vi "Test exp fit.vi"() -> ()   [LabVIEW 2020]
uses:
  controls/Color --typedef.ctl
  <vilib>/Utility/file.llb/Read Delimited Spreadsheet (DBL).vi
panel:
  out "MSE (red)":dbl
  out "MSE (green)":dbl
  out "MSE (blue)":dbl
  out "Red":cluster{dbl[], dbl[]}[](graph)
  out "Blue":cluster{dbl[], dbl[]}[](graph)
  out "Green":cluster{dbl[], dbl[]}[](graph)
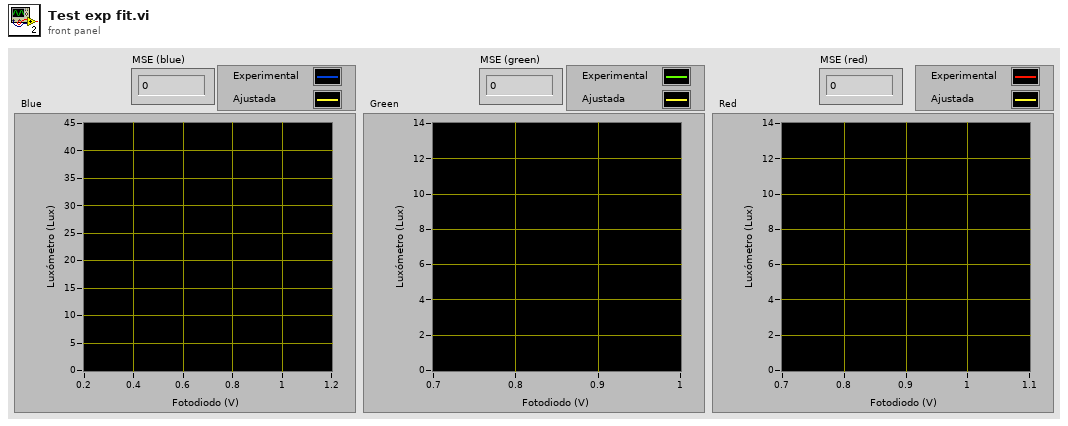
[diagram p1: front panel]
types:
  T1 = typedef "Color --typedef.ctl" = enum16{"Violeta (360-450nm)", "Azul (450-500nm)", "Verde(500-570nm)", "Amarillo (570-590nm)", "Naranja (600-610nm)", "Rojo (610-670nm)", "Blanco"}
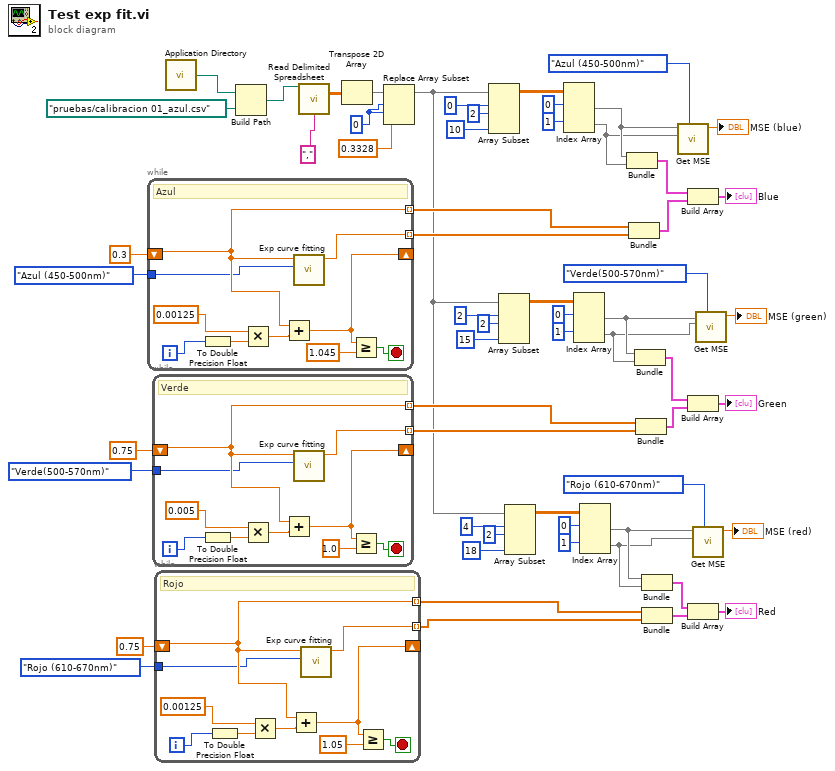
[diagram p0: block diagram]
diagram:
  w14 = 0 ("index (row)")
  n1 = while {
    shift-right: [w63] -> _
    shift-left: 0.3 -> [w62]
    tunnel: [w66] -> w55 mode=indexing
    tunnel: [w62] -> w54 mode=indexing
    tunnel: Color_--typedef."Azul (450-500nm)" ("Color 2") -> [w61]
    i -> [w70]
    stop <- w65 stop-if-true
    # "Azul"
    n2 = To Double Precision Float(number=w70) -> (double precision float=w69:dbl)
    n3 = Multiply(x=0.00125, y=w69) -> (x*y=w67:dbl)
    n4 = Add(x=w62, y=w67) -> (x+y=w63:dbl)
    n5 = call "Exp curve fitting.vi"("Color"=w61, "x (volts)"=w62) -> ("y (Lux)"=w66:dbl)  [unwired: 9 in]
    n6 = Greater Or Equal?(x=w63, y=1.045) -> (x >= y?=w65:bool)
  }
  n7 = while {
    shift-right: [w73] -> _
    shift-left: 0.75 -> [w72]
    tunnel: [w76] -> w58 mode=indexing
    tunnel: [w72] -> w59 mode=indexing
    tunnel: Color_--typedef."Verde(500-570nm)" ("Color") -> [w71]
    i -> [w80]
    stop <- w75 stop-if-true
    # "Verde"
    n8 = To Double Precision Float(number=w80) -> (double precision float=w79:dbl)
    n9 = Multiply(x=0.005, y=w79) -> (x*y=w77:dbl)
    n10 = Add(x=w72, y=w77) -> (x+y=w73:dbl)
    n11 = call "Exp curve fitting.vi"("Color"=w71, "x (volts)"=w72) -> ("y (Lux)"=w76:dbl)  [unwired: 9 in]
    n12 = Greater Or Equal?(x=w73, y=1.0) -> (x >= y?=w75:bool)
  }
  n13 = while {
    shift-right: [w83] -> _
    shift-left: 0.75 -> [w82]
    tunnel: [w86] -> w50 mode=indexing
    tunnel: [w82] -> w51 mode=indexing
    tunnel: Color_--typedef."Rojo (610-670nm)" ("Color 2") -> [w81]
    i -> [w90]
    stop <- w85 stop-if-true
    # "Rojo"
    n14 = To Double Precision Float(number=w90) -> (double precision float=w89:dbl)
    n15 = Multiply(x=0.00125, y=w89) -> (x*y=w87:dbl)
    n16 = Add(x=w82, y=w87) -> (x+y=w83:dbl)
    n17 = call "Exp curve fitting.vi"("Color"=w81, "x (volts)"=w82) -> ("y (Lux)"=w86:dbl)  [unwired: 9 in]
    n18 = Greater Or Equal?(x=w83, y=1.05) -> (x >= y?=w85:bool)
  }
  n19 = call <vilib>:"Application Directory.vi"() -> ("Application Directory"=w48:path)
  n20 = Build Path(base path=w48, name or relative path=path "pruebas/calibracion 01_azul.csv") -> (appended path=w46:path)
  n21 = call-poly <vilib>:"Read Delimited Spreadsheet.vi"("file path (dialog if empty)"=w46, "delimiter (\\t)"="," ("delimiter (\\t)")) -> ("all rows"=w16:dbl[][])  [unwired: 8 in, 5 out]
  n22 = Transpose 2D Array(2D array=w16) -> (transposed array=w20:dbl[][])
  n23 = Replace Array Subset(array=w20, new element=0.3328 ("new element/subarray"), index (row)=w14, index (col)=w14) -> (w15:dbl[][])
  n24 = Array Subset(array=w15, index (row)=0 ("index"), length (row)=2 ("length"), length (col)=10 ("length")) -> (w44:dbl[][])  [unwired: 1 in]
  n25 = Array Subset(array=w15, index (row)=2 ("index"), length (row)=2 ("length"), length (col)=15 ("length")) -> (w30:dbl[][])  [unwired: 1 in]
  n26 = Array Subset(array=w15, index (row)=4 ("index"), length (row)=2 ("length"), length (col)=18 ("length")) -> (w26:dbl[][])  [unwired: 1 in]
  n27 = Index Array(array=w44, index (row) #1=0 ("index (row)"), index (row) #2=1 ("index (row)")) -> (element #1=w12:dbl[], element #2=w8:dbl[])  [unwired: 2 in]
  n28 = Index Array(array=w30, index (row) #1=0 ("index (row)"), index (row) #2=1 ("index (row)")) -> (element #1=w9:dbl[], element #2=w7:dbl[])  [unwired: 2 in]
  n29 = Index Array(array=w26, index (row) #1=0 ("index (row)"), index (row) #2=1 ("index (row)")) -> (element #1=w3:dbl[], element #2=w2:dbl[])  [unwired: 2 in]
  n30 = Bundle(w12, w8) -> (w38:cluster{dbl[], dbl[]})  [unwired: 1 in]
  n31 = Bundle(w54, w55) -> (w37:cluster{dbl[], dbl[]})  [unwired: 1 in]
  n32 = Bundle(w9, w7) -> (w29:cluster{dbl[], dbl[]})  [unwired: 1 in]
  n33 = Bundle(w59, w58) -> (w28:cluster{dbl[], dbl[]})  [unwired: 1 in]
  n34 = Bundle(w3, w2) -> (w19:cluster{dbl[], dbl[]})  [unwired: 1 in]
  n35 = Bundle(w51, w50) -> (w18:cluster{dbl[], dbl[]})  [unwired: 1 in]
  n36 = call "Get MSE.vi"("Color"=Color_--typedef."Azul (450-500nm)", "y (lux)"=w8, "x (volts)"=w12) -> ("MSE"=→"MSE (blue)":dbl)  [unwired: 8 in]
  n37 = Build Array(w38, w37) -> (→"Blue":cluster{dbl[], dbl[]}[])
  n38 = Build Array(w29, w28) -> (→"Green":cluster{dbl[], dbl[]}[])
  n39 = Build Array(w19, w18) -> (→"Red":cluster{dbl[], dbl[]}[])
  n40 = call "Get MSE.vi"("Color"=Color_--typedef."Rojo (610-670nm)", "y (lux)"=w2, "x (volts)"=w3) -> ("MSE"=→"MSE (red)":dbl)  [unwired: 8 in]
  n41 = call "Get MSE.vi"("Color"=Color_--typedef."Verde(500-570nm)", "y (lux)"=w7, "x (volts)"=w9) -> ("MSE"=→"MSE (green)":dbl)  [unwired: 8 in]
